vi "header__e6e40d213d.vi"(0 "Frequency (Hz)":dbl, 1 "Frame Rate (fps)":string, 2 "Strain (%)":dbl, 3 "Binning":string, 4 "Gap (mm)":dbl, 5 "Phase Annulus":string, 6 "Initial position in Voltage (V)":dbl, 8 "Exposure (s)":dbl, 9 "Voltage to Displacement Constant (V/mm)":dbl, 10 "Sample":string, 11 "Temperature (oC)":string, 12 "Description":string, 13 "Objective:":string, 14 "Keywords":string, 15 "Camera":string, 16 "User":string, 17 "Numerical Aperture":string, 18 "Title of experiment":string) -> (20 "String":string)   [LabVIEW 2023]
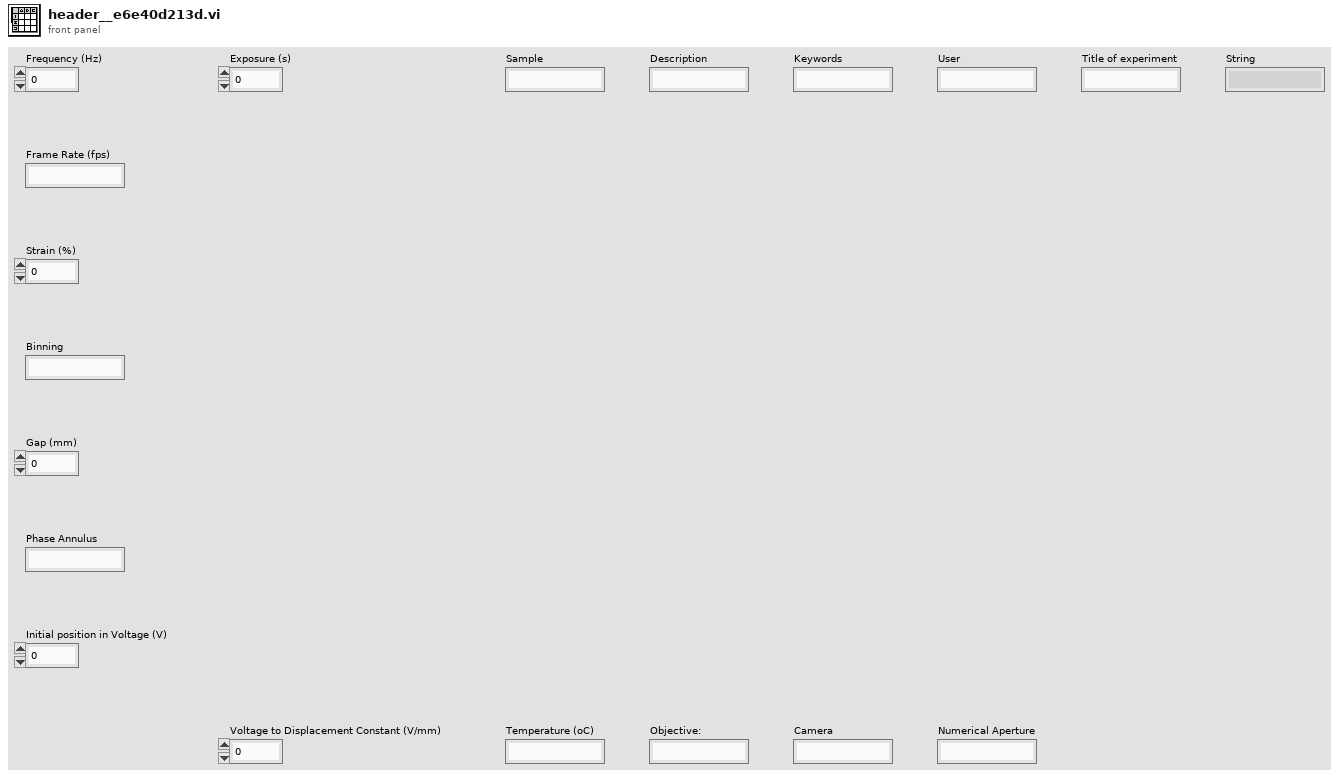
[diagram p1: front panel]
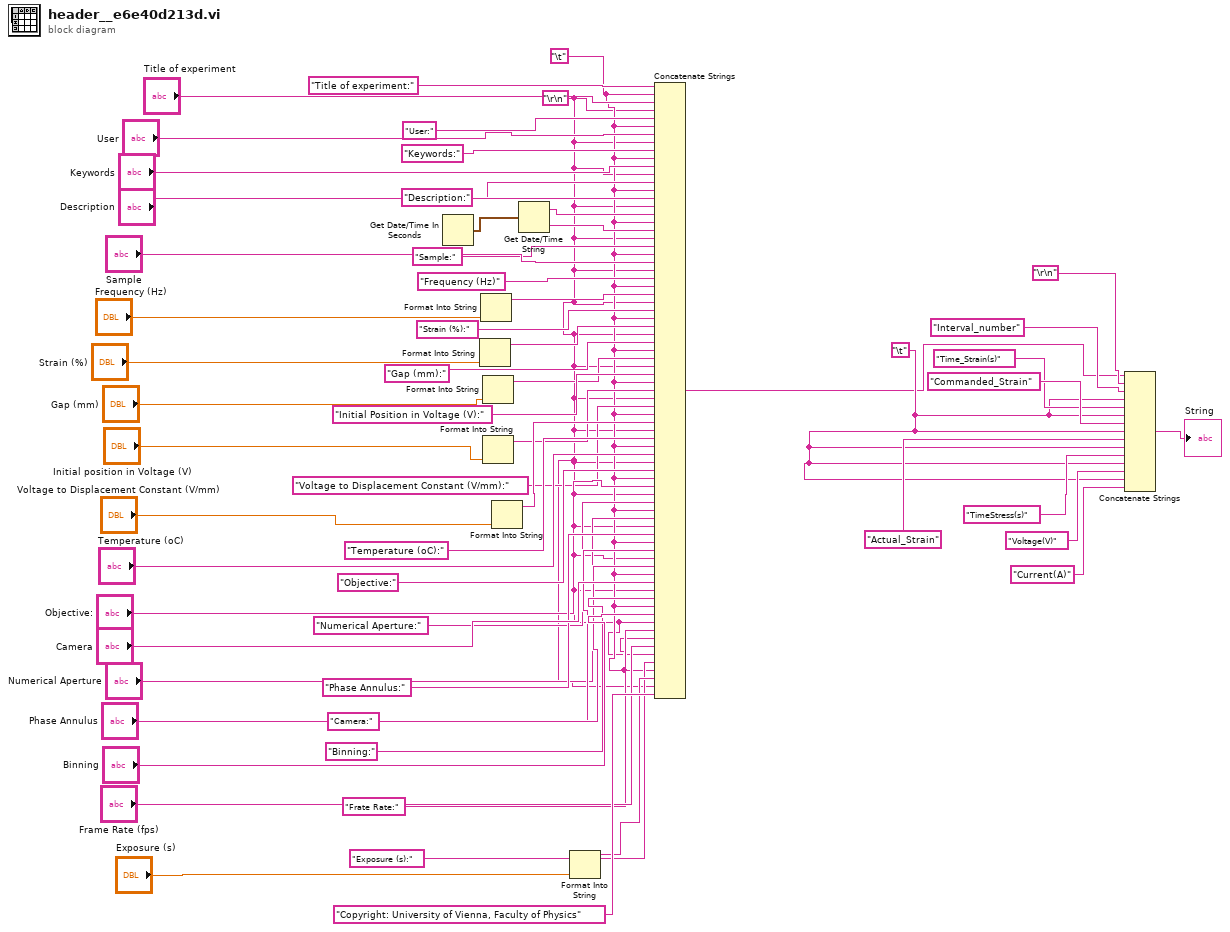
[diagram p0: block diagram]
diagram:
  w4 = "\t"
  w5 = "\r\n"
  w6 = "\t"
  n1 = Get Date/Time In Seconds() -> (seconds since 1Jan1904=w15:timestamp)
  n2 = Format Into String("Strain (%)") -> (resulting string=w25:string)  [unwired: 3 in, 1 out]
  n3 = Format Into String("Frequency (Hz)") -> (resulting string=w22:string)  [unwired: 3 in, 1 out]
  n4 = Format Into String("Gap (mm)") -> (resulting string=w28:string)  [unwired: 3 in, 1 out]
  n5 = Format Into String("Initial position in Voltage (V)") -> (resulting string=w31:string)  [unwired: 3 in, 1 out]
  n6 = Format Into String("Voltage to Displacement Constant (V/mm)") -> (resulting string=w33:string)  [unwired: 3 in, 1 out]
  n7 = Get Date/Time String(seconds (now)=w15) -> (date string=w16:string, time string=w17:string)  [unwired: 2 in]
  n8 = Format Into String("Exposure (s)") -> (resulting string=w56:string)  [unwired: 3 in, 1 out]
  n9 = Concatenate Strings("Title of experiment:", w6, "Title of experiment", w5, "User:", w6, "User", w5, "Keywords:", w6, "Keywords", w5, "Description:", w6, "Description", w5, w16, w6, w17, w5, "Sample:", w6, "Sample", w5, "Frequency (Hz)", w6, w22, w5, "Strain (%):", w6, w25, w5, "Gap (mm):", w6, w28, w5, "Initial Position in Voltage (V):", w6, w31, w5, "Voltage to Displacement Constant (V/mm):", w6, w33, w5, "Temperature (oC):", w6, "Temperature (oC)", w5, "Objective:", w6, "Objective:", w5, "Numerical Aperture:", w6, "Numerical Aperture", w5, "Phase Annulus:", w6, "Phase Annulus", w5, "Camera:", w6, "Camera", w5, "Binning:", w6, "Binning", w5, "Frate Rate:", w6, "Frame Rate (fps)", w5, "Exposure (s):", w6, w56, w5, "Copyright: University of Vienna, Faculty of Physics") -> (w1:string)
  n10 = Concatenate Strings(w1, "\r\n", "Interval_number", w4, "Time_Strain(s)", w4, "Commanded_Strain", w4, "Actual_Strain", w4, "TimeStress(s)", w4, "Voltage(V)", w4, "Current(A)") -> (→"String":string)
